vi "LABVIEW.vi"() -> ()   [LabVIEW 2021]
uses:
  <vilib>/Instr/_visa.llb/VISA Configure Serial Port (Instr).vi
panel:
  in  "?":bool
  in  "VISA resource name":refnum<visa-resource-name>
  in  "STOP":bool
  in  "Derecha":bool
  in  "Izquierda":bool
  in  "LED3":bool
  in  "LED2":bool
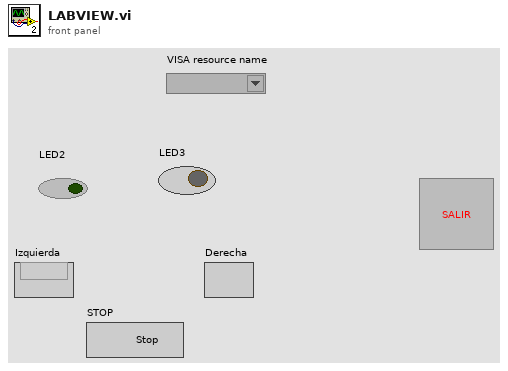
[diagram p1: front panel]
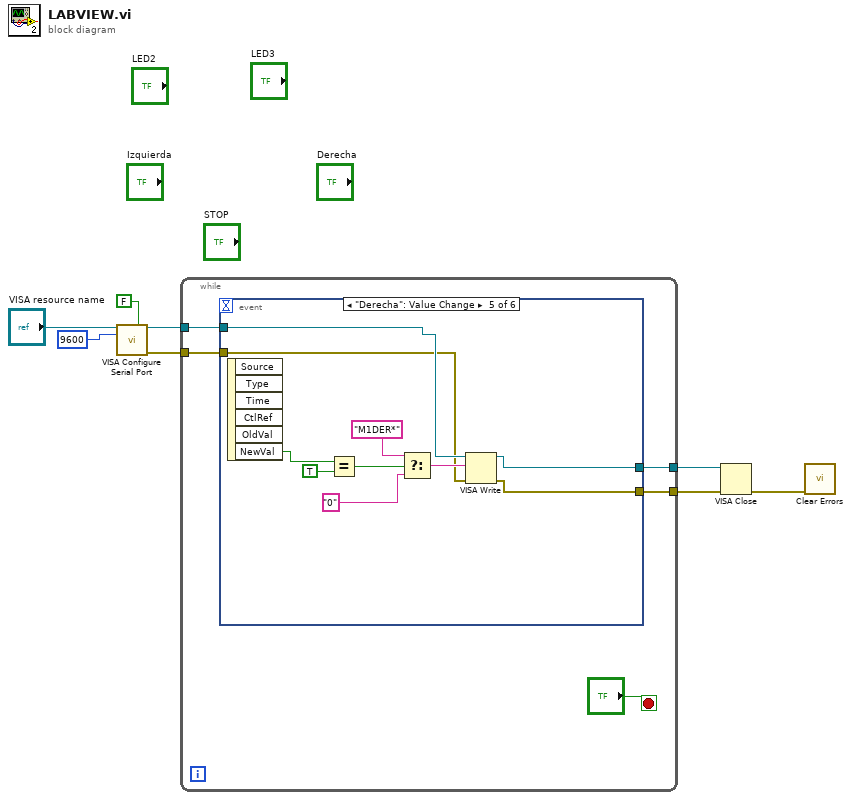
[diagram p0: block diagram]
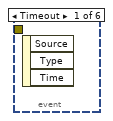
[diagram p2: hidden frame]
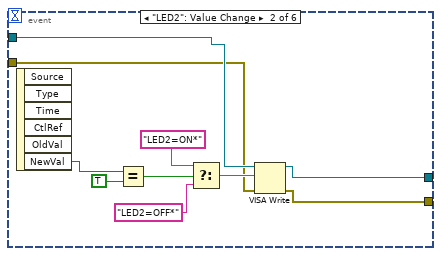
[diagram p3: hidden frame]
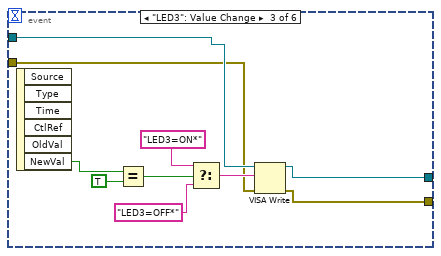
[diagram p4: hidden frame]
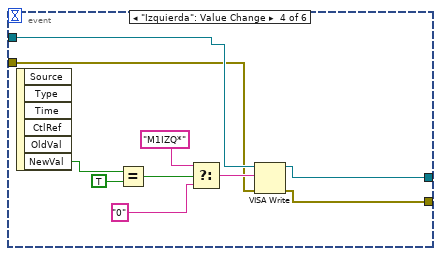
[diagram p5: hidden frame]
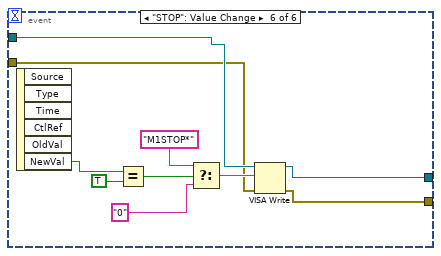
[diagram p6: hidden frame]
diagram:
  n1 = call-poly "VISA Configure Serial Port"("VISA resource name"="VISA resource name", "Enable Termination\nChar (T)"=FALSE ("Enable Termination\nChar (T)"), "baud rate (9600)"=u32 9600) -> ("VISA resource name out"=w5:refnum<visa-resource-name>, "error out"=w4:errorcluster)  [unwired: 11 in]
  n2 = while {
    tunnel: w5 -> [w12]
    tunnel: w4 -> [w11]
    tunnel: [w10] -> w3
    tunnel: [w9] -> w2
    stop <- "?" stop-if-true
    n3 = event shown="[4] \"Derecha\": Value Change" {
      selector: _ -> [_ _ _ _ _ _]
      dyn-events: _ -> [_ _ _ _ _ _]
      timeout: _ -> [_ _ _ _ _ _]
      tunnel: w12 -> [_ w17 w27 w37 w47 w57]
      tunnel: w11 -> [_ w16 w26 w36 w46 w56]
      tunnel: [_ w15 w25 w35 w45 w55] -> w10
      tunnel: [_ w14 w24 w34 w44 w54] -> w9
      event Timeout {
        n4 = event-data() -> ()  [unwired: 1 in, 3 out]
      }
      event "LED2": Value Change {
        n5 = event-data() -> ("NewVal"=w23:bool)  [unwired: 1 in, 5 out]
        n6 = Equal?(x=w23, y=TRUE) -> (x = y?=w21:bool)
        n7 = Select(t="LED2=ON*", s=w21, f="LED2=OFF*") -> (s? t:f=w18:string)
        n8 = VISA Write(VISA resource name=w17, write buffer=w18, error in (no error)=w16) -> (VISA resource name out=w15:refnum<visa-resource-name>, error out=w14:errorcluster)  [unwired: 1 out]
      }
      event "LED3": Value Change {
        n9 = event-data() -> ("NewVal"=w33:bool)  [unwired: 1 in, 5 out]
        n10 = Equal?(x=w33, y=TRUE) -> (x = y?=w31:bool)
        n11 = Select(t="LED3=ON*", s=w31, f="LED3=OFF*") -> (s? t:f=w28:string)
        n12 = VISA Write(VISA resource name=w27, write buffer=w28, error in (no error)=w26) -> (VISA resource name out=w25:refnum<visa-resource-name>, error out=w24:errorcluster)  [unwired: 1 out]
      }
      event "Izquierda": Value Change {
        n13 = event-data() -> ("NewVal"=w43:bool)  [unwired: 1 in, 5 out]
        n14 = Equal?(x=w43, y=TRUE) -> (x = y?=w41:bool)
        n15 = Select(t="M1IZQ*", s=w41, f="0") -> (s? t:f=w38:string)
        n16 = VISA Write(VISA resource name=w37, write buffer=w38, error in (no error)=w36) -> (VISA resource name out=w35:refnum<visa-resource-name>, error out=w34:errorcluster)  [unwired: 1 out]
      }
      event "Derecha": Value Change {
        n17 = event-data() -> ("NewVal"=w53:bool)  [unwired: 1 in, 5 out]
        n18 = Equal?(x=w53, y=TRUE) -> (x = y?=w51:bool)
        n19 = Select(t="M1DER*", s=w51, f="0") -> (s? t:f=w48:string)
        n20 = VISA Write(VISA resource name=w47, write buffer=w48, error in (no error)=w46) -> (VISA resource name out=w45:refnum<visa-resource-name>, error out=w44:errorcluster)  [unwired: 1 out]
      }
      event "STOP": Value Change {
        n21 = event-data() -> ("NewVal"=w63:bool)  [unwired: 1 in, 5 out]
        n22 = Equal?(x=w63, y=TRUE) -> (x = y?=w61:bool)
        n23 = Select(t="M1STOP*", s=w61, f="0") -> (s? t:f=w58:string)
        n24 = VISA Write(VISA resource name=w57, write buffer=w58, error in (no error)=w56) -> (VISA resource name out=w55:refnum<visa-resource-name>, error out=w54:errorcluster)  [unwired: 1 out]
      }
    }
  }
  n25 = VISA Close(VISA resource name=w3, error in (no error)=w2) -> (error out=w1:errorcluster)
  n26 = call <vilib>:"Clear Errors.vi"("error in (no error)"=w1) -> ()  [unwired: 5 in, 2 out]
